vi "SeqEditor_ParamMousehit.vi"(8 "Coords":T1, 11 "MulticolumnListbox in":refnum<vi>) -> ()   [LabVIEW 2017, in "NLTest.lvclass"]
uses:
  NLTest.lvclass
  <vilib>/Utility/miscctls.llb/LVPoint32TypeDef.ctl
  SeqEditor_Global.vi
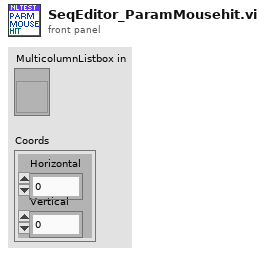
[diagram p1: front panel]
types:
  T1 = typedef "LVPoint32TypeDef.ctl" = cluster{"Horizontal":i32, "Vertical":i32}
  T2 = typedef "LVRowAndColumnTypeDef.ctl" = cluster{"Row":i32, "Column":i32}
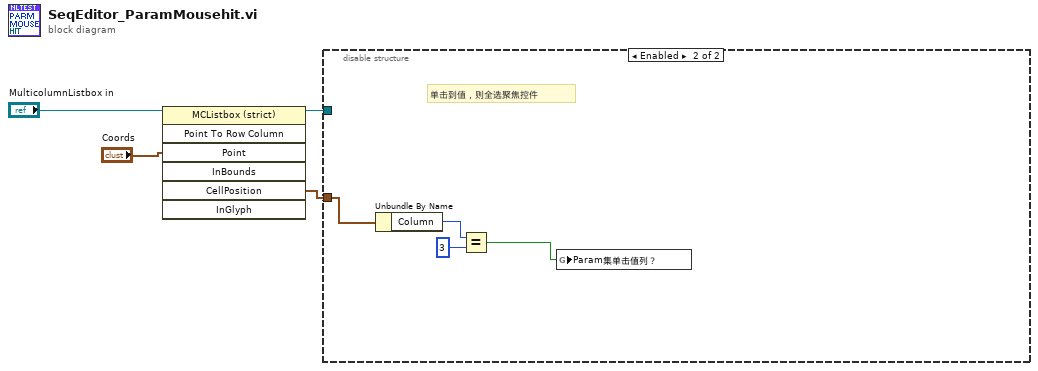
[diagram p0: block diagram]
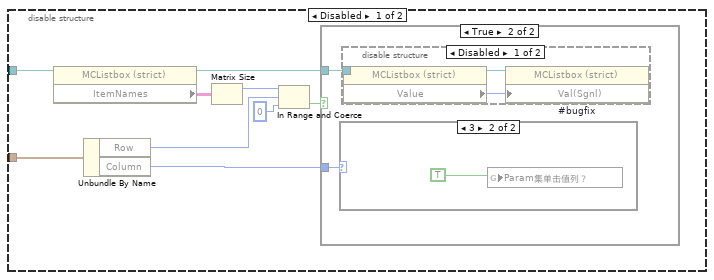
[diagram p2: hidden frame]
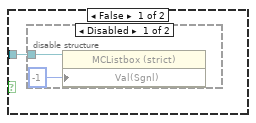
[diagram p3: hidden frame]
diagram:
  n1 = invoke class="MCListbox (strict)" method="Point To Row Column"(reference="MulticolumnListbox in", "Point"="Coords") -> (reference out=w3:refnum<vi>, "CellPosition"=w4:T2)  [unwired: 5 in, 5 out]
  n2 = disable-structure shown="Enabled" {
    disable-tunnel: w4 -> [w12 w26]
    disable-tunnel: w3 -> [w6 _]
    frame Disabled {
      n3 = property class="MCListbox (strict)"(reference=w6) -> (reference out=w11:refnum<vi>, "ItemNames"=w7:string[][])  [unwired: 1 in, 1 out]
      n4 = Unbundle By Name(w12) -> ("Row"=w13:i32, "Column"=w5:i32)
      n5 = Matrix Size(0:w7) -> (1:w8:i32)  [unwired: 1 out]
      n6 = In Range and Coerce(upper limit=w8, x=w13, lower limit=0) -> (In Range?=w10:bool)  [unwired: 1 out]
      n7 = case shown="True" w10 {
        tunnel: w11 -> [w14 w17]
        tunnel: w5 -> [_ w18]
        frame False {
          n8 = disable-structure shown="Disabled" {
            disable-tunnel: w14 -> [w16 _]
            frame Disabled {
              n9 = property class="MCListbox (strict)"(reference=w16, "Val(Sgnl)"=-1 ("Value (Signaling)")) -> ()  [unwired: 1 in, 2 out]
            }
            frame Enabled {
            }
          }
        }
        frame True {
          n10 = case shown="3" w18 {
            frame 0, Default {
            }
            frame 3 {
              n11 = global write "SeqEditor_Global.vi" "Param集单击值列？"(TRUE ("Parmcol2hit")) -> ()
            }
          }
          n12 = disable-structure shown="Disabled" {
            disable-tunnel: w17 -> [w21 _]
            frame Disabled {
              n13 = property class="MCListbox (strict)"(reference=w21) -> (reference out=w20:refnum<vi>, "Value"=w19:i32)  [unwired: 1 in, 1 out]
              n14 = property on="#bugfix" class="MCListbox (strict)"(reference=w20, "Val(Sgnl)"=w19) -> ()  [unwired: 1 in, 2 out]
            }
            frame Enabled {
            }
          }
        }
      }
    }
    frame Enabled {
      # "单击到值，则全选聚焦控件"
      n15 = Unbundle By Name(w26) -> ("Column"=w25:i32)
      n16 = Equal?(x=w25, y=3) -> (x = y?=w23:bool)
      n17 = global write "SeqEditor_Global.vi" "Param集单击值列？"(w23) -> ()
    }
  }
